vi "TCP Sender.vi"() -> ()   [LabVIEW 2026]
panel:
  in  "OK Button":bool
  out "error out":errorcluster
  out "Port":dbl
  out "Address":string
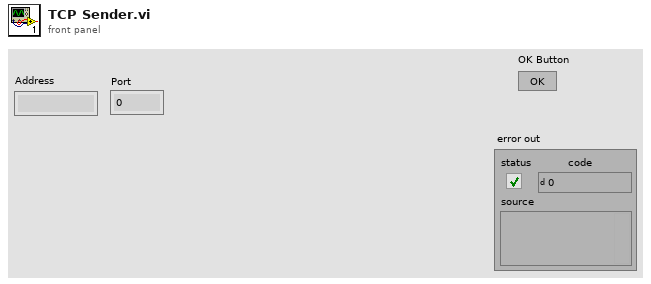
[diagram p1: front panel]
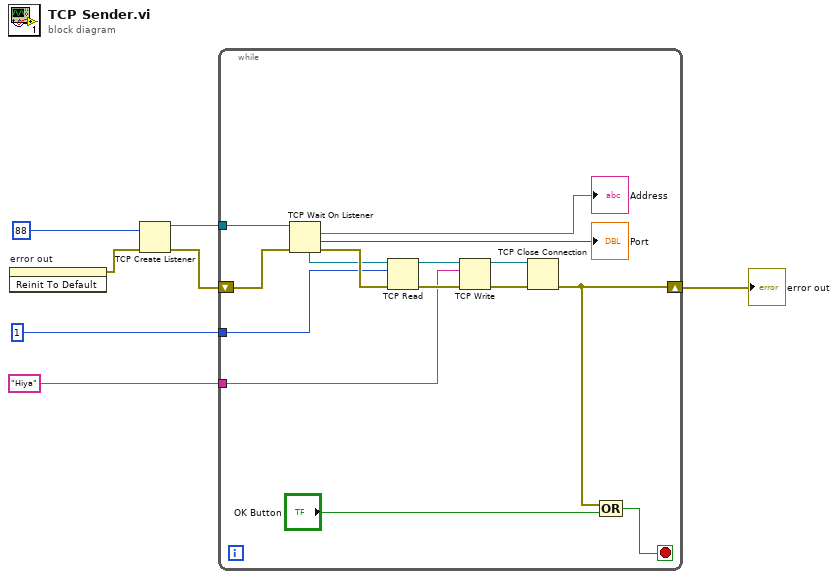
[diagram p0: block diagram]
diagram:
  n1 = invoke on="error out" class="Clust (strict)" method="Reinit To Default"() -> (error out=w2:errorcluster)  [unwired: 3 in, 2 out]
  n2 = TCP Create Listener(8:w2, 10:88) -> (0:w5:errorcluster, 3:w6:refnum<k5>)  [unwired: 3 in, 1 out]
  n3 = while {
    tunnel: w6 -> [w22]
    shift-right: [w9] -> w1
    shift-left: w5 -> [w19]
    tunnel: 1 -> [w16]
    tunnel: "Hiya" -> [w13]
    stop <- w8 stop-if-true
    n4 = TCP Wait On Listener(8:w19, 11:w22) -> (0:w18:errorcluster, 1:→"Port":u16, 2:→"Address":string, 4:w17:refnum<k5>)  [unwired: 2 in, 1 out]
    n5 = TCP Read(connection ID=w17, bytes to read=w16, error in (no error)=w18) -> (connection ID out=w14:refnum<k5>, error out=w15:errorcluster)  [unwired: 2 in, 1 out]
    n6 = TCP Write(connection ID=w14, data in=w13, error in (no error)=w15) -> (connection ID out=w11:refnum<k5>, error out=w12:errorcluster)  [unwired: 1 in, 1 out]
    n7 = TCP Close Connection(connection ID=w11, error in (no error)=w12) -> (error out=w9:errorcluster)  [unwired: 1 in, 1 out]
    n8 = Compound Arithmetic op=OR(w9, "OK Button") -> (w8:bool)
  }
  "error out" <- w1
